vi "Test Day Rollup.vi"(8 "error in":errorcluster, 10 "Work Folder":path, 11 "Test Data Folder":path) -> (0 "error out":errorcluster, 2 "Report":string, 3 "Passed":bool)   [LabVIEW 2026]
doc: "Tests Day Rollup.vi with the Project Store of the schema-v2 sample data (Test Data\\Samples, copied into a new case folder) and nine entries built here on 2025-10-06, given out of order. Checks: four entries of one task become one row (6 rows in all); Hours rounds to the nearest quarter hour (1 h 07 m -> 1.00, 1 h 08 m -> 1.25, 1 h 07 m 30 s -> 1.25, 5 min -> 0.00, 2 h 53 m -> 3.00); Descriptions skip an empty and a repeated description and keep start-time order; a running entry (End Time 0) counts up to Now; rows are ordered by first start time; project names are looked up by ID and an unknown Project ID is shown as the ID; Row Copy Text is each row's Descriptions; All Copy Text is TAB-separated with rows joined by CR LF; an empty Day Entries gives empty outputs and no error.\n\nInputs: Test Data Folder; Work Folder; error in. Outputs: Passed; Report; error out.\n\nGenerated by: Claude"
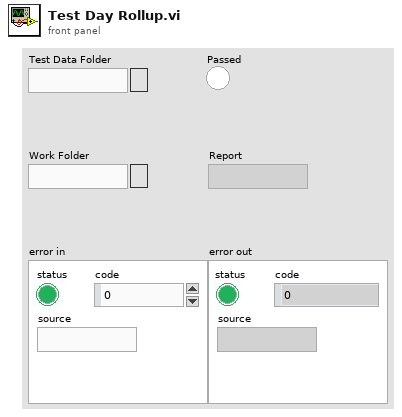
[diagram p1: front panel]
types:
  T1 = cluster{"ID":string, "Project ID":string, "Task ID":string, "Start Time":timestamp, "End Time":timestamp, "Description":string}[]
  T2 = cluster{"ID":string, "Project ID":string, "Task ID":string, "Start Time":timestamp, "End Time":timestamp, "Description":string}
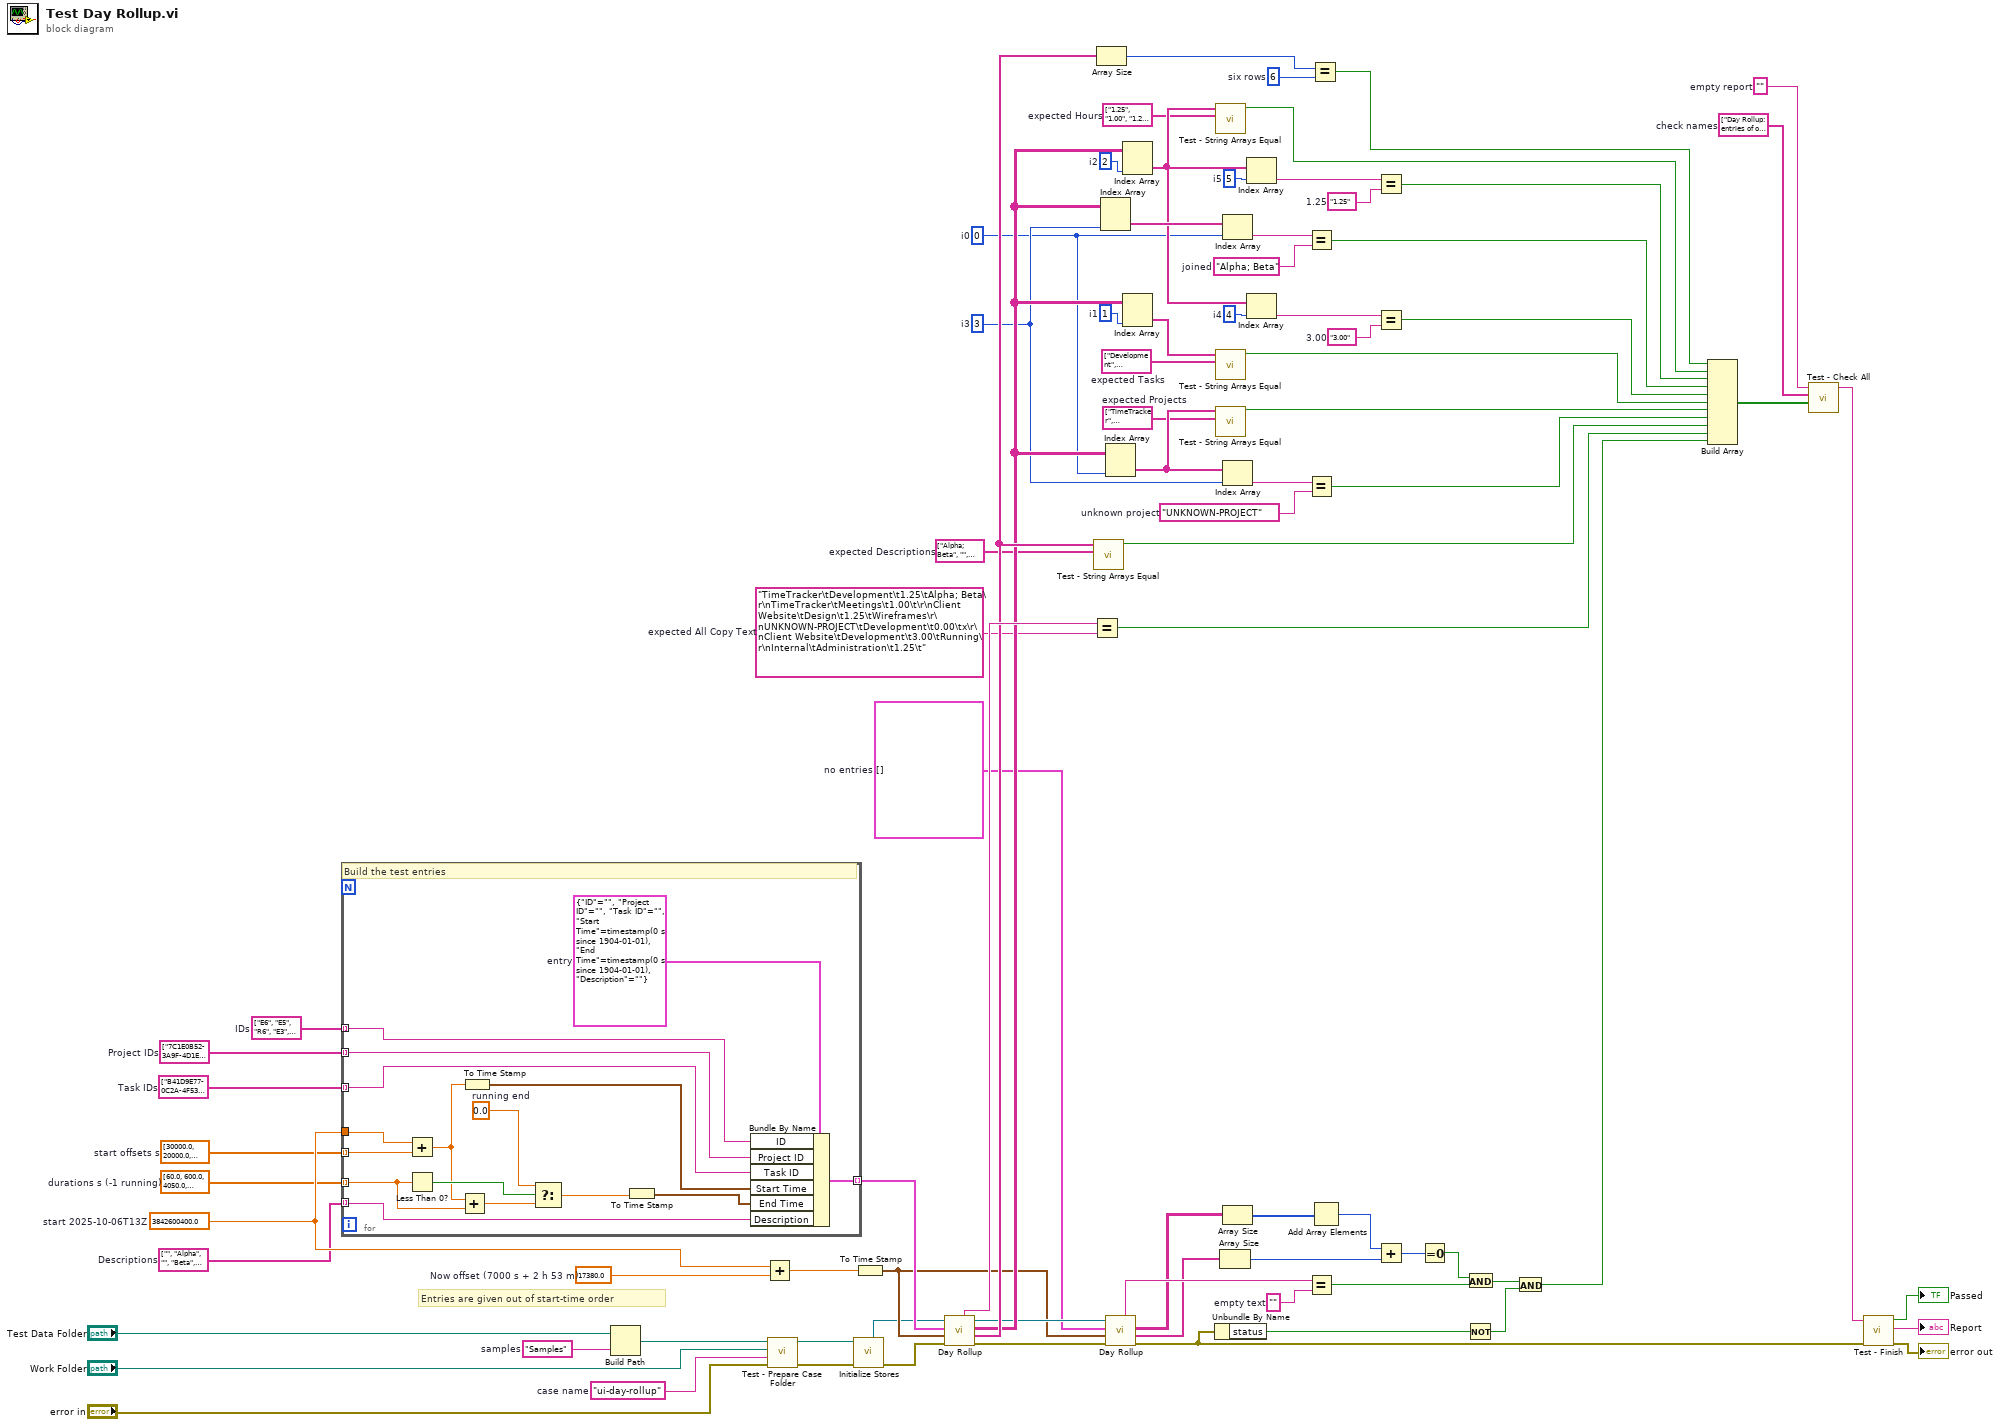
[diagram p0: block diagram]
diagram:
  w36 = string[] ["Day Rollup: entries of one task add up to one row (6 rows)", "Day Rollup: Hours rounds to the quarter hour (1.25 1.00 1.25 0.00 3.00 1.25)", "Day Rollup: 1 h 07 m 30 s rounds up to 1.25", "Day Rollup: Descriptions skip empty and repeated text in start order", "Day Rollup: running entry is counted up to Now (2 h 53 m = 3.00)", "Day Rollup: rows are ordered by first start time", "Day Rollup: names by ID and an unknown Project ID shown as the ID", "Day Rollup: unknown Project ID row shows UNKNOWN-PROJECT", "Day Rollup: Row Copy Text is each row's Descriptions", "Day Rollup: All Copy Text is TAB-separated with CR LF between rows", "Day Rollup: empty Day Entries gives empty outputs and no error"]  # check names
  w35 = ""  # empty text
  w34 = "TimeTracker\tDevelopment\t1.25\tAlpha; Beta\r\nTimeTracker\tMeetings\t1.00\t\r\nClient Website\tDesign\t1.25\tWireframes\r\nUNKNOWN-PROJECT\tDevelopment\t0.00\tx\r\nClient Website\tDevelopment\t3.00\tRunning\r\nInternal\tAdministration\t1.25\t"  # expected All Copy Text
  w33 = "UNKNOWN-PROJECT"  # unknown project
  w32 = "3.00"  # 3.00
  w31 = "1.25"  # 1.25
  w30 = "Alpha; Beta"  # joined
  w29 = string[] ["Alpha; Beta", "", "Wireframes", "x", "Running", ""]  # expected Descriptions
  w28 = string[] ["TimeTracker", "TimeTracker", "Client Website", "UNKNOWN-PROJECT", "Client Website", "Internal"]  # expected Projects
  w27 = string[] ["Development", "Meetings", "Design", "Development", "Development", "Administration"]  # expected Tasks
  w26 = string[] ["1.25", "1.00", "1.25", "0.00", "3.00", "1.25"]  # expected Hours
  w25 = 6  # six rows
  w24 = 5  # i5
  w23 = 4  # i4
  w22 = 1  # i1
  w21 = 3  # i3
  w20 = 2  # i2
  w19 = 0  # i0
  w18 = T1 []  # no entries
  w17 = 17380.0  # Now offset (7000 s + 2 h 53 m)
  w16 = 3842600400.0  # start 2025-10-06T13Z
  w15 = string[] ["", "Alpha", "", "Beta", "Running", "x", "Wireframes", "", "Alpha"]  # Descriptions
  w14 = dbl[] [60.0, 600.0, 4050.0, 420.0, -1.0, 300.0, 4080.0, 4020.0, 3600.0]  # durations s (-1 running)
  w13 = dbl[] [30000.0, 20000.0, 8000.0, 10000.0, 7000.0, 6000.0, 5000.0, 4000.0, 0.0]  # start offsets s
  w12 = string[] ["B41D9E77-0C2A-4F53-8E16-5A9D3C7B2E04", "B41D9E77-0C2A-4F53-8E16-5A9D3C7B2E04", "3F5E8C21-D4B7-4A09-B6E2-5C1A7D9F0E84", "B41D9E77-0C2A-4F53-8E16-5A9D3C7B2E04", "14B9E6D3-A07C-4D52-9F18-3E6A5C2B8D70", "B41D9E77-0C2A-4F53-8E16-5A9D3C7B2E04", "8E2D5A47-1B6C-4F90-8D3A-7C4B0E9F2A16", "F03C6B1E-2D79-4C85-A4E0-9B5D8A1C3E67", "B41D9E77-0C2A-4F53-8E16-5A9D3C7B2E04"]  # Task IDs
  w11 = string[] ["7C1E0B52-3A9F-4D1E-9B7A-2F6C8D4E1A90", "7C1E0B52-3A9F-4D1E-9B7A-2F6C8D4E1A90", "E91B7D34-5C0A-4B8F-9E26-1D7A3F5C8B42", "7C1E0B52-3A9F-4D1E-9B7A-2F6C8D4E1A90", "2A6F4C18-9D3B-4E7A-A1C5-8B0E6D2F4A73", "UNKNOWN-PROJECT", "2A6F4C18-9D3B-4E7A-A1C5-8B0E6D2F4A73", "7C1E0B52-3A9F-4D1E-9B7A-2F6C8D4E1A90", "7C1E0B52-3A9F-4D1E-9B7A-2F6C8D4E1A90"]  # Project IDs
  w10 = string[] ["E6", "E5", "R6", "E3", "R5", "R4", "R3", "R2", "E1"]  # IDs
  w9 = ""  # empty report
  w8 = "ui-day-rollup"  # case name
  w7 = "Samples"  # samples
  # "Entries are given out of start-time order"
  n1 = for {
    tunnel: w10 -> [w85] mode=indexing
    tunnel: w11 -> [w86] mode=indexing
    tunnel: w12 -> [w87] mode=indexing
    tunnel: w13 -> [w88] mode=indexing
    tunnel: w14 -> [w89] mode=indexing
    tunnel: w15 -> [w90] mode=indexing
    tunnel: w16 -> [w91]
    tunnel: [w100] -> w44 mode=indexing
    w93 = 0.0  # running end
    w92 = T2 {"ID"="", "Project ID"="", "Task ID"="", "Start Time"=timestamp(0 s since 1904-01-01), "End Time"=timestamp(0 s since 1904-01-01), "Description"=""}  # entry
    # "Build the test entries"
    n2 = Add(x=w91, y=w88) -> (x+y=w94:dbl)
    n3 = Less Than 0?(x=w89) -> (x < 0?=w96:bool)
    n4 = Add(x=w94, y=w89) -> (x+y=w95:dbl)
    n5 = To Time Stamp(1:w94) -> (0:w98:timestamp)
    n6 = Select(t=w93, s=w96, f=w95) -> (s? t:f=w97:dbl)
    n7 = To Time Stamp(1:w97) -> (0:w99:timestamp)
    n8 = Bundle By Name(cluster=w92, "ID"=w85, "Project ID"=w86, "Task ID"=w87, "Start Time"=w98, "End Time"=w99, "Description"=w90) -> (w100:T2)
  }
  n9 = Build Path(base path="Test Data Folder", name or relative path=w7) -> (appended path=w37:path)
  n10 = Add(x=w16, y=w17) -> (x+y=w42:dbl)
  n11 = call "Test - Prepare Case Folder.vi"("error in (no error)"="error in", "Case Name"=w8, "Work Folder"="Work Folder", "Source Folder"=w37) -> ("error out"=w38:errorcluster, "Case Folder"=w39:path)  [unwired: 6 in]
  n12 = call "Initialize Stores.vi"("error in"=w38, "Data Folder"=w39) -> ("error out"=w40:errorcluster, "Project Store out"=w41:refnum<class "Project Store.lvclass">)  [unwired: 5 in, 3 out]
  n13 = To Time Stamp(1:w42) -> (0:w43:timestamp)
  n14 = call "Day Rollup.vi"("error in"=w40, "Now"=w43, "Day Entries"=w44, "Project Store in"=w41) -> ("error out"=w49:errorcluster, "Row Copy Text"=w47:string[], "Rollup Rows"=w46:string[][], "Project Store out"=w45:refnum<class "Project Store.lvclass">, "All Copy Text"=w48:string)  [unwired: 3 in]
  n15 = Equal?(x=w48, y=w34) -> (x = y?=w72:bool)
  n16 = call "Test - String Arrays Equal.vi"("Expected"=w29, "Actual"=w47) -> ("Equal?"=w71:bool)  [unwired: 8 in, 1 out]
  n17 = Array Size(array=w47) -> (size(s)=w54:i32)
  n18 = Index Array(array=w46, index (col)=w21) -> (element=w59:string[])  [unwired: 1 in]
  n19 = Index Array(array=w46, index (col)=w19) -> (element=w58:string[])  [unwired: 1 in]
  n20 = call "Day Rollup.vi"("error in"=w49, "Now"=w43, "Day Entries"=w18, "Project Store in"=w45) -> ("error out"=w53:errorcluster, "Row Copy Text"=w51:string[], "Rollup Rows"=w50:string[][], "All Copy Text"=w52:string)  [unwired: 3 in, 1 out]
  n21 = Index Array(array=w46, index (col)=w20) -> (element=w56:string[])  [unwired: 1 in]
  n22 = Index Array(array=w46, index (col)=w22) -> (element=w57:string[])  [unwired: 1 in]
  n23 = Unbundle By Name(w53) -> ("status"=w79:bool)
  n24 = call "Test - String Arrays Equal.vi"("Expected"=w26, "Actual"=w56) -> ("Equal?"=w60:bool)  [unwired: 8 in, 1 out]
  n25 = call "Test - String Arrays Equal.vi"("Expected"=w27, "Actual"=w57) -> ("Equal?"=w67:bool)  [unwired: 8 in, 1 out]
  n26 = call "Test - String Arrays Equal.vi"("Expected"=w28, "Actual"=w58) -> ("Equal?"=w68:bool)  [unwired: 8 in, 1 out]
  n27 = Array Size(array=w51) -> (size(s)=w75:i32)
  n28 = Index Array(array=w59, index=w19) -> (element=w63:string)
  n29 = Index Array(array=w58, index=w21) -> (element=w69:string)
  n30 = Array Size(array=w50) -> (size(s)=w73:i32[])
  n31 = Index Array(array=w56, index=w24) -> (element=w61:string)
  n32 = Index Array(array=w56, index=w23) -> (element=w65:string)
  n33 = Equal?(x=w63, y=w30) -> (x = y?=w64:bool)
  n34 = Equal?(x=w69, y=w33) -> (x = y?=w70:bool)
  n35 = Equal?(x=w52, y=w35) -> (x = y?=w78:bool)
  n36 = Equal?(x=w54, y=w25) -> (x = y?=w55:bool)
  n37 = Add Array Elements(numeric array=w73) -> (sum=w74:i32)
  n38 = Equal?(x=w61, y=w31) -> (x = y?=w62:bool)
  n39 = Equal?(x=w65, y=w32) -> (x = y?=w66:bool)
  n40 = Add(x=w74, y=w75) -> (x+y=w76:i32)
  n41 = Equal To 0?(x=w76) -> (x = 0?=w77:bool)
  n42 = Not(x=w79) -> (.not. x?=w80:bool)
  n43 = And(x=w77, y=w78) -> (x .and. y?=w81:bool)
  n44 = And(x=w81, y=w80) -> (x .and. y?=w82:bool)
  n45 = Build Array(w55, w60, w62, w64, w66, w67, w68, w70, w71, w72, w82) -> (w83:bool[])
  n46 = call "Test - Check All.vi"("Conditions"=w83, "Check Names"=w36, "Report in"=w9) -> ("Report out"=w84:string)  [unwired: 7 in, 1 out]
  n47 = call "Test - Finish.vi"("error in (no error)"=w53, "Report"=w84) -> ("error out"=→"error out":errorcluster, "Report out"=→"Report":string, "Passed"=→"Passed":bool)  [unwired: 7 in]
